vi "FuncVI-vhShow.vi"(5 "InstanceRef":T2, 9 "arg list":T1[](array[typedef])) -> (0 "error out":bool, 3 "result":T1)   [LabVIEW 2021]
doc: "::: CalcExpress Toolkit :::\nCopyright (c) 2000-2026 Konstantin Shifershteyn. All rights reserved."
uses:
  cetypes.llb/CalcExpress Function Argument Info.ctl
  cetypes.llb/CalcExpress Instance RefNum.ctl
panel:
  in  "max arg num":i32=4
  in  "min arg num":i32=1
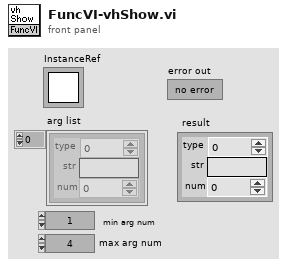
[diagram p1: front panel]
types:
  T1 = typedef "CalcExpress Function Argument Info.ctl" = cluster{"type":u32, "str":string, "num":dbl}
  T2 = typedef "CalcExpress Instance RefNum.ctl" = refnum<k1>
  T3 = cluster{"index":i32, "data type":enum32{"String", "DBL Number", "identifier", "1D Array of DBL", "2D Array of DBL", "CDB Number", "1D Array of CDB", "2D Array of CDB", "1D Array of String", "2D Array of String", "Unknown data type"}, "default num":dbl, "default str":string}[]
  T4 = cluster{"index":i32, "data type":enum32{"String", "DBL Number", "identifier", "1D Array of DBL", "2D Array of DBL", "CDB Number", "1D Array of CDB", "2D Array of CDB", "1D Array of String", "2D Array of String", "Unknown data type"}, "default num":dbl, "default str":string}
  T5 = cluster{"data type":enum32{"String", "DBL Number", "identifier", "1D Array of DBL", "2D Array of DBL", "CDB Number", "1D Array of CDB", "2D Array of CDB", "1D Array of String", "2D Array of String", "Unknown data type"}, "str":string, "num":dbl}
  T6 = typedef "VarMan Variable Context Handle.ctl" = i32
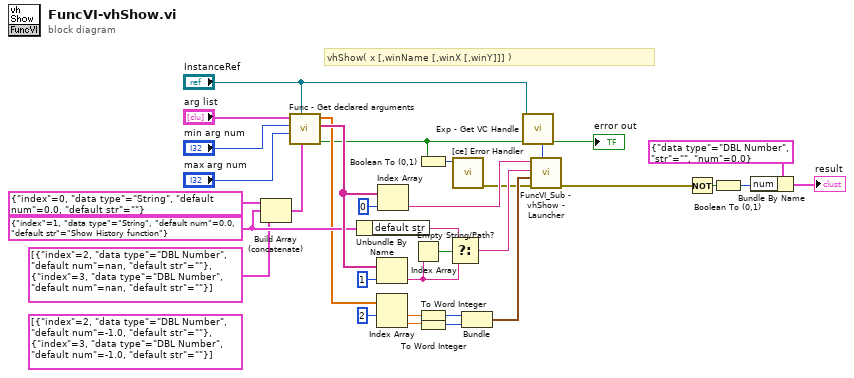
[diagram p0: block diagram]
diagram:
  (unwired) T3 [{"index"=2, "data type"=enum."DBL Number", "default num"=-1.0, "default str"=""}, {"index"=3, "data type"=enum."DBL Number", "default num"=-1.0, "default str"=""}]
  w26 = T4 {"index"=1, "data type"=enum."String", "default num"=0.0, "default str"="Show History function"} ("arg descriptor")
  # "vhShow( x [,winName [,winX [,winY]]] )"
  n1 = Build Array (concatenate)(T4 {"index"=0, "data type"=enum."String", "default num"=0.0, "default str"=""} ("arg descriptor"), w26, T3 [{"index"=2, "data type"=enum."DBL Number", "default num"=nan, "default str"=""}, {"index"=3, "data type"=enum."DBL Number", "default num"=nan, "default str"=""}]) -> (w33:T3)
  n2 = call "Func - Get declared arguments.vi"("arg descriptors"=w33, "InstanceRef"="InstanceRef", "max arg num"="max arg num", "min arg num"="min arg num", "arg list"="arg list") -> ("error out"=w3:bool, "str list"=w30:string[], "num list"=w19:dbl[])  [unwired: 3 in, 1 out]
  n3 = Unbundle By Name(w26) -> ("default str"=w27:string)
  n4 = Index Array(array=w30, index=1) -> (element=w29:string)
  n5 = Index Array(array=w19, index #1=2) -> (element #1=w18:dbl, element #2=w2:dbl)  [unwired: 1 in]
  n6 = Index Array(array=w30, index=0) -> (element=w8:string)
  n7 = Empty String/Path?(string/path=w29) -> (empty?=w28:bool)
  n8 = Boolean To (0,1)(Boolean=w3) -> (0, 1=w5:i16)
  n9 = To Word Integer(number=w18) -> (16bit integer=w17:i16)
  n10 = To Word Integer(number=w2) -> (16bit integer=w16:i16)
  n11 = Select(t=w27, s=w28, f=w29) -> (s? t:f=w25:string)
  n12 = call "[ce] Error Handler.vi"("error code"=w5) -> ("error out"=w4:errorcluster)  [unwired: 9 in, 1 out]
  n13 = Bundle(w17, w16) -> (w7:cluster{i16, i16})  [unwired: 1 in]
  n14 = call "Exp - Get VC Handle.vi"("error in"=w3, "InstanceRef"="InstanceRef") -> ("error out"=→"error out":bool, "VC Handle"=w11:T6)  [unwired: 4 in, 2 out]
  n15 = call "FuncVI_Sub - vhShow - Launcher.vi"("VC Handle"=w11, "error in"=w4, "left-top corner"=w7, "win name"=w25, "var name"=w8) -> ("error out"=w1:errorcluster)  [unwired: 6 in]
  n16 = Not(x=w1) -> (.not. x?=w13:bool)
  n17 = Boolean To (0,1)(Boolean=w13) -> (0, 1=w24:i16)
  n18 = Bundle By Name(cluster=T5 {"data type"=enum."DBL Number", "str"="", "num"=0.0} ("opd info"), "num"=w24) -> (→"result":T5)
